vi "Detect Steering Misalignment.vi"(11 "Motors In":T1 {"Steer Scaling" format="%.2f"; "Drive Scaling" format="%.2f"; "Pod Locations (ft)"."Right Back" format="%.2f"; "Pod Locations (ft)"."Right Front" format="%.2f"; "Pod Locations (ft)"."Left Back" format="%.2f"; "Pod Locations (ft)"."Left Front" format="%.2f"}) -> (3 "Motors out":T1 {"Steer Scaling" format="%.2f"; "Drive Scaling" format="%.2f"; "Pod Locations (ft)"."Right Back" format="%.2f"; "Pod Locations (ft)"."Right Front" format="%.2f"; "Pod Locations (ft)"."Left Back" format="%.2f"; "Pod Locations (ft)"."Left Front" format="%.2f"})   [LabVIEW 2023]
uses:
  <vilib>/Analysis/NI_AAL_Angle.lvlib
  <vilib>/Analysis/coordinate.llb/Wrap Angle (scalar).vi
  <vilib>/Analysis/coordinate.llb/Angle Units.ctl
  5e800f26-b426-49e4-b681-eb18440e8622.vi
  <vilib>/Rock Robotics/Network Tables/NT Read String.vi
  <resource>/objmgr/REVSpark.rc
  <vilib>/MRC/MrcLib.lvlib
  <vilib>/Rock Robotics/Network Tables/NT Write Boolean.vi
  swerve-template/Type Definitions/Data/Pod Positions.ctl
  <vilib>/REV Custom Controls/REVSparkRefnum.ctl
  <vilib>/REVLibDriver/REVLibDriver.lvlib
  swerve-template/Type Definitions/Hardware/Swerve Drives/(NEO-NEO-ThroughBore-Pigeon2) Swerve.ctl
panel:
  out "Array":dbl[](array[numeric])
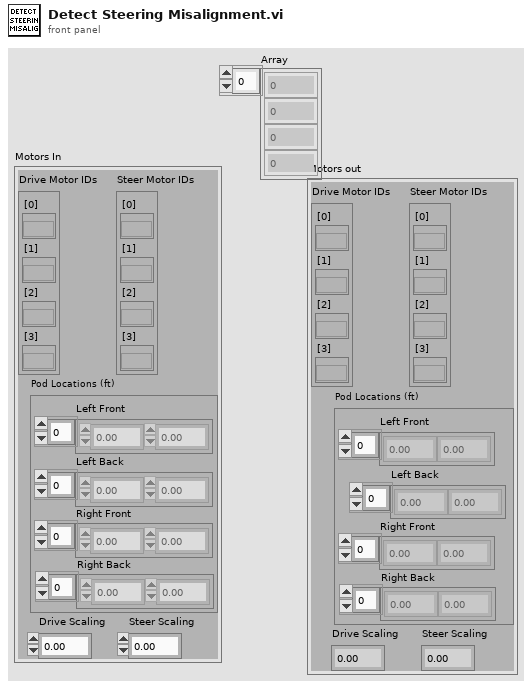
[diagram p1: front panel]
types:
  T1 = typedef "(NEO-NEO-ThroughBore-Pigeon2) Swerve.ctl" = cluster{"Drive Motor IDs":cluster{"[0]":T2, "[1]":T2, "[2]":T2, "[3]":T2}, "Steer Motor IDs":cluster{"[0]":T2, "[1]":T2, "[2]":T2, "[3]":T2}, "Pod Locations (ft)":T3, "Drive Scaling":dbl, "Steer Scaling":dbl}
  T2 = typedef "REVLibDriver.lvlib/REVSparkRefnum.ctl" = refnum<k20>
  T3 = typedef "Pod Positions.ctl" = cluster{"Left Front":dbl[], "Left Back":dbl[], "Right Front":dbl[], "Right Back":dbl[]}
  T4 = typedef "NI_AAL_Angle.lvlib/Angle Units.ctl" = i32
  T5 = cluster{"Left Front":dbl, "Left Back":dbl, "Right Front":dbl, "Right Back":dbl}
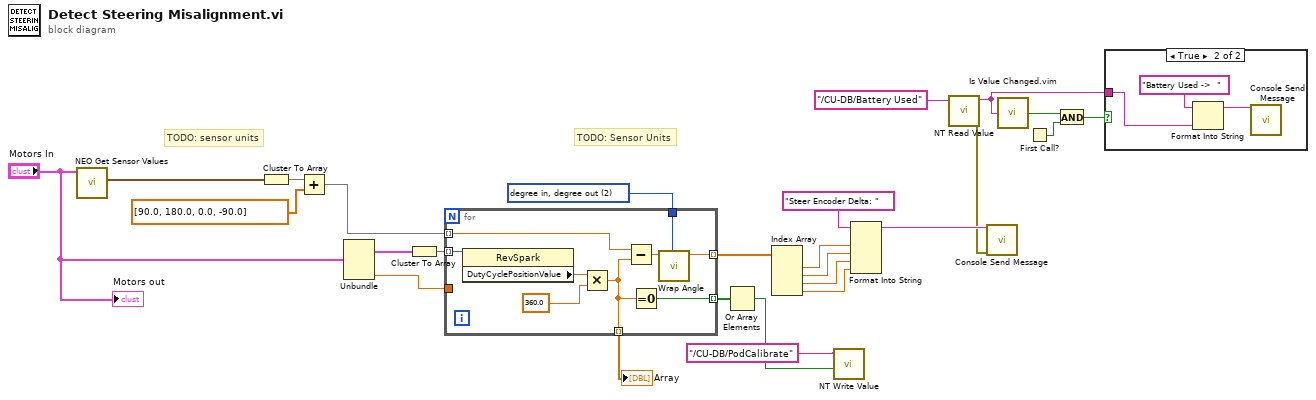
[diagram p0: block diagram]
diagram:
  w26 = T4 2 items=["radian in, radian out", "radian in, degree out", "degree in, degree out", "degree in, radian out"] ("angle units")
  # "TODO: Sensor Units"
  # "TODO: sensor units"
  n1 = call "NEO Get Sensor Values.vi"("Motors In"="Motors In") -> ("Steer Angles (degrees)"=w20:T5)  [unwired: 9 in, 1 out]
  n2 = Cluster To Array(cluster=w20) -> (array=w23:dbl[])
  n3 = Add(x=w23, y=dbl[] [90.0, 180.0, 0.0, -90.0]) -> (x+y=w21:dbl[])
  n4 = Unbundle("Motors In") -> ("Steer Motor IDs"=w24:cluster{"[0]":T2, "[1]":T2, "[2]":T2, "[3]":T2}, "Steer Scaling"=w2:dbl)  [unwired: 3 out]
  n5 = Cluster To Array(cluster=w24) -> (array=w25:T2[])
  n6 = for {
    tunnel: w25 -> [w30] mode=indexing
    tunnel: w21 -> [w35] mode=indexing
    tunnel: w26 -> [w33]
    tunnel: [w32] -> w13 mode=indexing
    tunnel: [w31] -> w7 mode=indexing
    tunnel: w2 -> [_]
    tunnel: [w28] -> w1 mode=indexing
    n7 = property class="RevSpark"(reference=w30) -> ("DutyCyclePositionValue"=w29:sgl)  [unwired: 1 in, 2 out]
    n8 = Multiply(x=w29, y=sgl 360.0) -> (x*y=w28:sgl)
    n9 = Subtract(x=w35, y=w28) -> (x-y=w34:dbl)
    n10 = Equal To 0?(x=w28) -> (x = 0?=w31:bool)
    n11 = call-poly <vilib>:"Wrap Angle.vi"("angle units"=w33, "angle in"=w34) -> ("angle out"=w32:dbl)  [unwired: 8 in, 1 out]
  }
  "Array" <- w1
  n12 = Or Array Elements(Boolean array=w7) -> (logical OR=w6:bool)
  n13 = Index Array(array=w13) -> (element #1=w17:dbl, element #2=w16:dbl, element #3=w15:dbl, element #4=w14:dbl)  [unwired: 4 in]
  n14 = call-poly <vilib>:"NT Write Value.vi"("value"=w6, "name"="/CU-DB/PodCalibrate") -> ()  [unwired: 9 in, 1 out]
  n15 = Format Into String(initial string="Steer Encoder Delta: ", w17, w16, w15, w14) -> (resulting string=w4:string)  [unwired: 2 in, 1 out]
  n16 = call-poly <vilib>:"NT Read Value.vi"("name"="/CU-DB/Battery Used") -> ("error out"=w3:errorcluster, "value"=w11:string)  [unwired: 8 in, 1 out]
  n17 = call <vilib>:"Console Send Message.vi"("Message"=w4, "error in (no error)"=w3) -> ()  [unwired: 13 in, 1 out]
  n18 = call "Is Value Changed.vim"("value"=w11) -> ("changed or first call?"=w10:bool)
  n19 = First Call?() -> (First Call?: T/F=w8:bool)
  n20 = And(x=w10, y=w8) -> (x .and. y?=w9:bool)
  n21 = case shown="True" w9 {
    tunnel: w11 -> [_ w37]
    frame False {
    }
    frame True {
      n22 = Format Into String(initial string="Battery Used ->  ", w37) -> (resulting string=w36:string)  [unwired: 2 in, 1 out]
      n23 = call <vilib>:"Console Send Message.vi"("Message"=w36) -> ()  [unwired: 14 in, 1 out]
    }
  }
  "Motors out" <- "Motors In"
